vi "Get Arguments as LabVIEW Data.vi"(7 "type":variant, 8 "error in (no error)":errorcluster, 11 "Call in":refnum<class "Call.lvclass">) -> (0 "error out":errorcluster, 2 "LabVIEW Data":variant, 3 "Call out":refnum<class "Call.lvclass">)   [LabVIEW 2020, in "jki_python_bridge.lvlib" / "Call.lvclass"]
uses:
  Call.lvclass
  Python Data Tools/source/Python String to LabVIEW Data/Python String to LabVIEW Data (Variant).vi
  Call.lvclass/Call.ctl
  Python Data Tools/source/jki_python_data_tools.lvlib
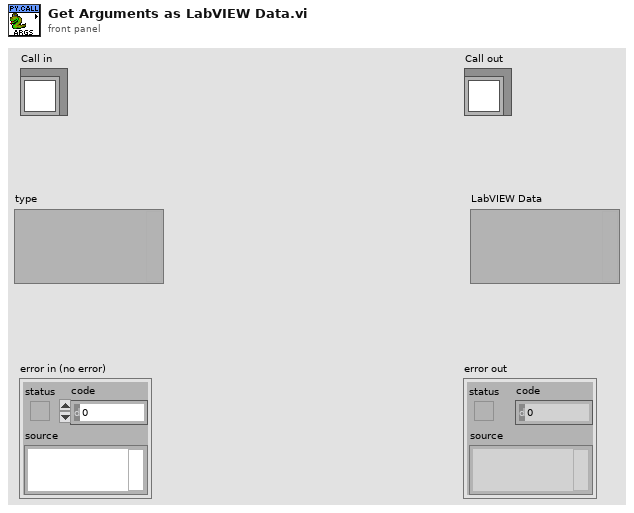
[diagram p1: front panel]
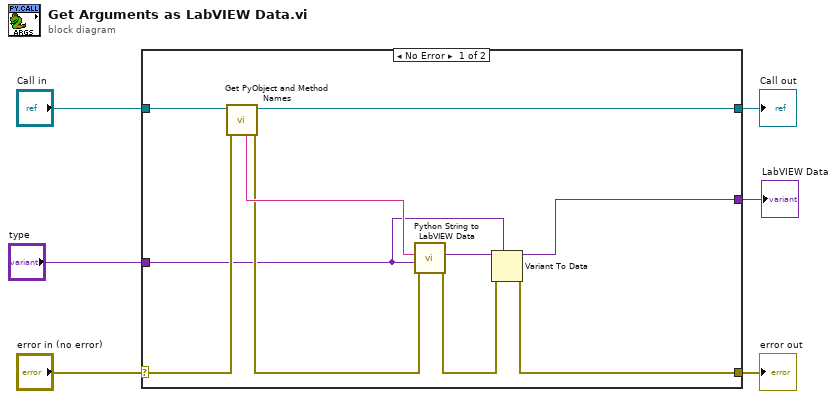
[diagram p0: block diagram]
diagram:
  n1 = case shown="No Error" "error in (no error)" {
    selector: "error in (no error)" -> [w13 w18]
    tunnel: [w7 w18] -> w5
    tunnel: [w15 w17] -> w3
    tunnel: "Call in" -> [w16 w17]
    tunnel: [w9 _] -> w2
    tunnel: "type" -> [w11 _]
    frame No Error {
      n2 = call "Get PyObject and Method Names.vi"("error in (no error)"=w13, "Call in"=w16) -> ("error out"=w12:errorcluster, "Call out"=w15:refnum<class "Call.lvclass">, "Arguments String"=w14:string)  [unwired: 5 in, 2 out]
      n3 = call-poly "Python String to LabVIEW Data.vi"("error in (no error)"=w12, "type"=w11, "Python String"=w14) -> ("error out"=w8:errorcluster, "LabVIEW Data"=w10:variant)  [unwired: 7 in]
      n4 = Variant To Data(error in=w8, type=w11, Variant=w10) -> (data=w9:variant, error out=w7:errorcluster)
    }
    frame Error {
    }
  }
  "error out" <- w5
  "Call out" <- w3
  "LabVIEW Data" <- w2
